vi "SUP_SyncTap.vi"(5 "source_vi":refnum<vi>) -> (0 "telemetry error":errorcluster caption="sortie d'erreur")   [LabVIEW 2012]
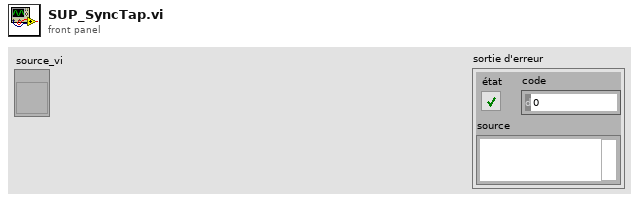
[diagram p1: front panel]
types:
  T1 = cluster{string, "Get Control Value Variant":variant, "error out":errorcluster}
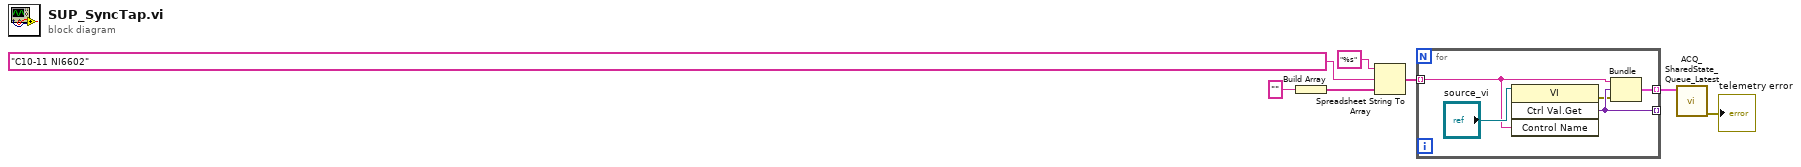
[diagram p0: block diagram]
diagram:
  n1 = Build Array("") -> (w6:string[])
  n2 = Spreadsheet String To Array(format string="%s" ("chaîne de format"), spreadsheet string="C10-11 NI6602" ("chaîne de type tableur"), array type (2D Dbl)=w6) -> (array=w4:string[])  [unwired: 1 in]
  n3 = for {
    tunnel: w4 -> [w11] mode=indexing
    tunnel: [w10] -> _ mode=indexing
    tunnel: [w8] -> w3 mode=indexing
    n4 = invoke class="VI" method="Ctrl Val.Get"(reference="source_vi", "Control Name"=w11) -> (error out=w9:errorcluster, "Get Control Value Variant"=w10:variant)  [unwired: 2 in, 2 out]
    n5 = Bundle(w11, "Get Control Value Variant"=w10, "error out"=w9) -> (w8:T1)  [unwired: 1 in]
  }
  n6 = call "ACQ_SharedState_Queue_Latest.vi"("packet"=w3) -> ("telemetry error"=→"telemetry error":errorcluster)  [unwired: 9 in, 1 out]
